vi "Generate Transformation Matrix.vi"(8 "error in":errorcluster, 11 "Referential in":refnum<class "Referential.lvclass">) -> (0 "error out":errorcluster, 2 "Matrix Array":cluster{"A x B":T1}[](array[cluster]), 3 "Referential out":refnum<class "Referential.lvclass">)   [LabVIEW 2019, in "Referential.lvclass"]
uses:
  Referential.lvclass
  <vilib>/Analysis/Matrix/Datatypes/RealMatrix.ctl
  <vilib>/Analysis/Matrix/NI_Matrix.lvlib
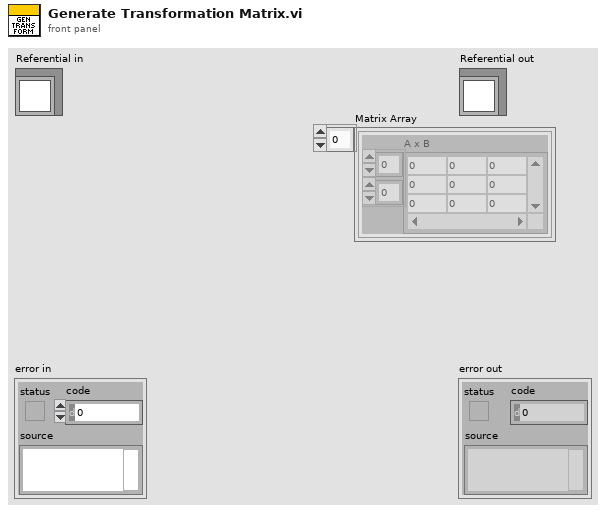
[diagram p1: front panel]
types:
  T1 = typedef "NI_Matrix.lvlib/RealMatrix.ctl" = dbl[][]
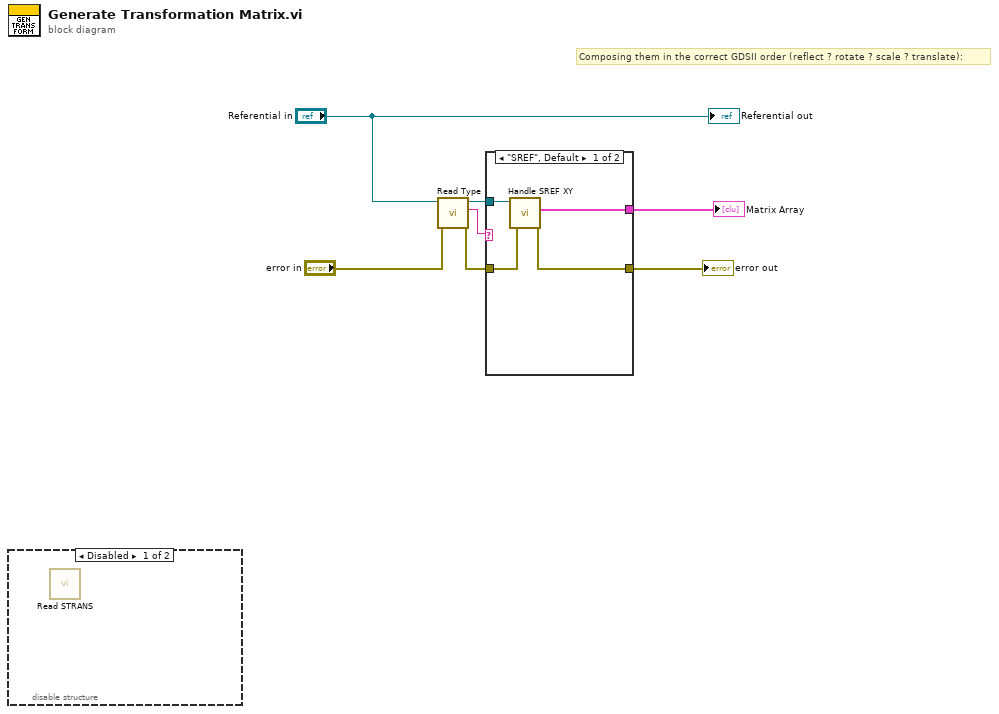
[diagram p0: block diagram]
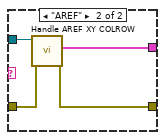
[diagram p2: hidden frame]
diagram:
  # "Composing them in the correct GDSII order (reflect ? rotate ? scale ? translate):"
  n1 = disable-structure shown="Disabled" {
    frame Disabled {
      n2 = call-dynamic "Read STRANS.vi"() -> ()  [unwired: 9 in, 3 out]
    }
    frame Enabled {
    }
  }
  n3 = call-dynamic "Read Type.vi"("error in (no error)"="error in", "Element in"="Referential in") -> ("error out"=w2:errorcluster, "Type"=w5:string, "Element out"=w6:refnum<class "Referential.lvclass">)  [unwired: 7 in]
  n4 = case shown="\"SREF\", Default" w5 {
    tunnel: [w10 w14] -> w4
    tunnel: w6 -> [w11 w15]
    tunnel: w2 -> [w8 w13]
    tunnel: [w9 w12] -> w1
    frame "SREF", Default {
      n5 = call "Handle SREF XY.vi"("error in"=w8, "Referential in"=w11) -> ("error out"=w9:errorcluster, "Transformation"=w10:cluster{"XY Matrix":T1}[])  [unwired: 7 in, 1 out]
    }
    frame "AREF" {
      n6 = call "Handle AREF XY COLROW.vi"("error in"=w13, "Referential in"=w15) -> ("error out"=w12:errorcluster, "XY Vectors"=w14:cluster{"XY Matrix":T1}[])  [unwired: 7 in, 1 out]
    }
  }
  "error out" <- w1
  "Matrix Array" <- w4
  "Referential out" <- "Referential in"
